vi "Documentation Application Tool.vi"() -> ()   [LabVIEW 2016]
uses:
  <vilib>/ni/Tree/Tree Manager/Tree.lvclass
  States.ctl
  <vilib>/ni/Tree/Data Types/String/String.lvclass/String.ctl
  <vilib>/ni/Tree/Data Types/String/To String Tree Data.vi
  <vilib>/ni/Tree/Data Types/String/From String Tree Data.vi
  <vilib>/ni/Tree/Data Types/String/String.lvclass
  C:/Program Files/National Instruments/LabVIEW 2016/vi.lib/ni/Tree/Tree Data/Tree Data.lvclass
  <vilib>/ni/Tree/Tree Manager/API/Set Meta Data.vi
  <vilib>/ni/Tree/Tree Manager/API/Set Attribute.vi
  <vilib>/ni/Tree/Tree Manager/API/Get Name.vi
  <vilib>/ni/Tree/Tree Manager/API/Set Name.vi
  <vilib>/ni/Tree/Tree Manager/API/Set Attribute Tree Data.vi
  <vilib>/xml/Load XML File.vi
  <vilib>/ni/Tree/Tree Manager/API/List Roots.vi
  <vilib>/ni/Tree/Tree Manager/API/Get Attribute Tree Data.vi
  <vilib>/ni/Tree/Tree Manager/API/Get Meta Data.vi
  <vilib>/ni/Tree/Tree Manager/API/Delete Attribute Tree Data.vi
  <vilib>/ni/Tree/Tree Manager/API/List Attribute Names.vi
  <vilib>/ni/Tree/Tree Manager/API/Get Attribute.vi
  <vilib>/xml/NI_XML.lvlib
panel:
  in  "Load XML File":bool
  in  "XML File Path":path=path "C:/Git/rfic-reference-design-libraries-csharp/CodeReport.xml"
  in  "Load Search Directory":bool
  in  "Search Directory":path=path "C:/Git/rf-adv-reference-design-libraries-labview/Source/SG"
  in  "Code Modules":string(tree)
  in  "XML File":string(tree)
  out "Selected Element":string
  in  "Element Description":string
  in  "Copy":bool
  out "Selected XML Data":string
  in  "Cancel":bool
  in  "Apply All Unsaved":bool
  in  "Cancel All":bool
  in  "Apply":bool
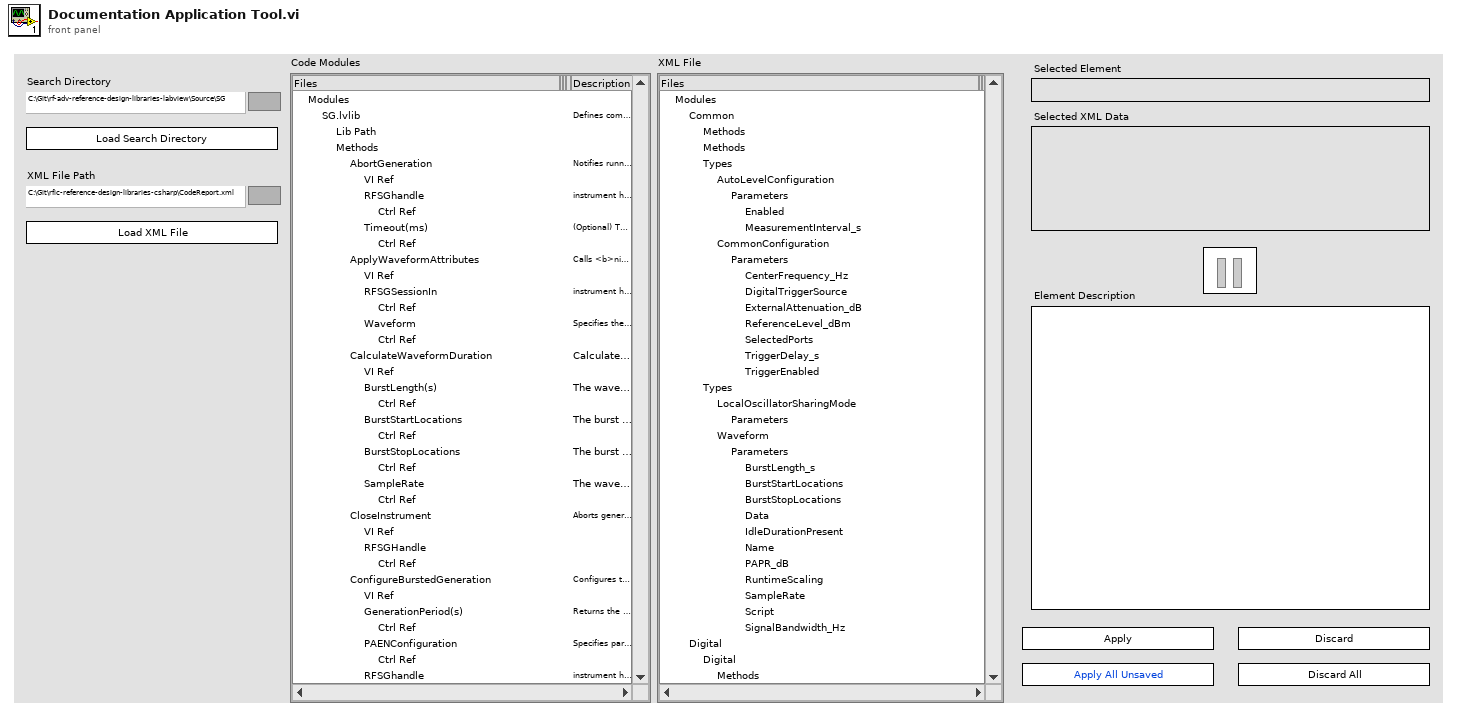
[diagram p1: front panel]
types:
  T1 = typedef "States.ctl" = enum16{"<Init>", "Wait for Event", "Update Code Modules Display", "Save Files", "<Shutdown>"}
  T2 = cluster{"LabVIEW Tree":refnum<data-value>, "XML Tree":refnum<data-value>, "References":refnum<vi>[], "Unsaved Items":variant, "Control Strings":string[], "Items to Save":string[]}
  T3 = enum32{"invalid VI type", "Standard VI", "Control VI", "Global VI", "Polymorphic VI", "Configuration VI", "SubSystem", "Facade VI", "Method VI", "Statechart Diagram VI"}
  T4 = enum16{"Left Button", "Center Button", "Right Button", "Window Close"}
  T5 = typedef "eventvkey.ctl" = enum16{"ASCII", "Enter", "Return", "Shift", "Ctrl", "Alt", "Cmd", "Opt", "Caps", "NumLock", "Clear", "Break", "Up", "Down", "Left", "Right", "Insert", "Delete", "Home", "End", "PageUp", "PageDown", "Escape", "Help", "Pause", "ScrollLock", "F1", "F2", "F3", "F4", "F5", "F6", "F7", "F8", "F9", "F10", "F11", "F12", "F13", "F14", "F15", "F16", "F17", "F18", "F19", "F20", "F21", "F22", "F23", "F24", "Play", "VolumeUp", "VolumeDown", "Mute", "Two Byte Char"}
  T6 = cluster{"Shift":bool, "Ctrl":bool, "Alt":bool, "Cmd":bool, "Opt":bool}
  T7 = cluster{"Left Cell String":string, "Child Text":string[], "Child Tag":string, "Item Indent":i32, "Child Only?":bool, "Glyph Index":i32}[]
  T8 = typedef "LVNodeAndColumnTypeDef.ctl" = cluster{"Node":string, "Column":i32}
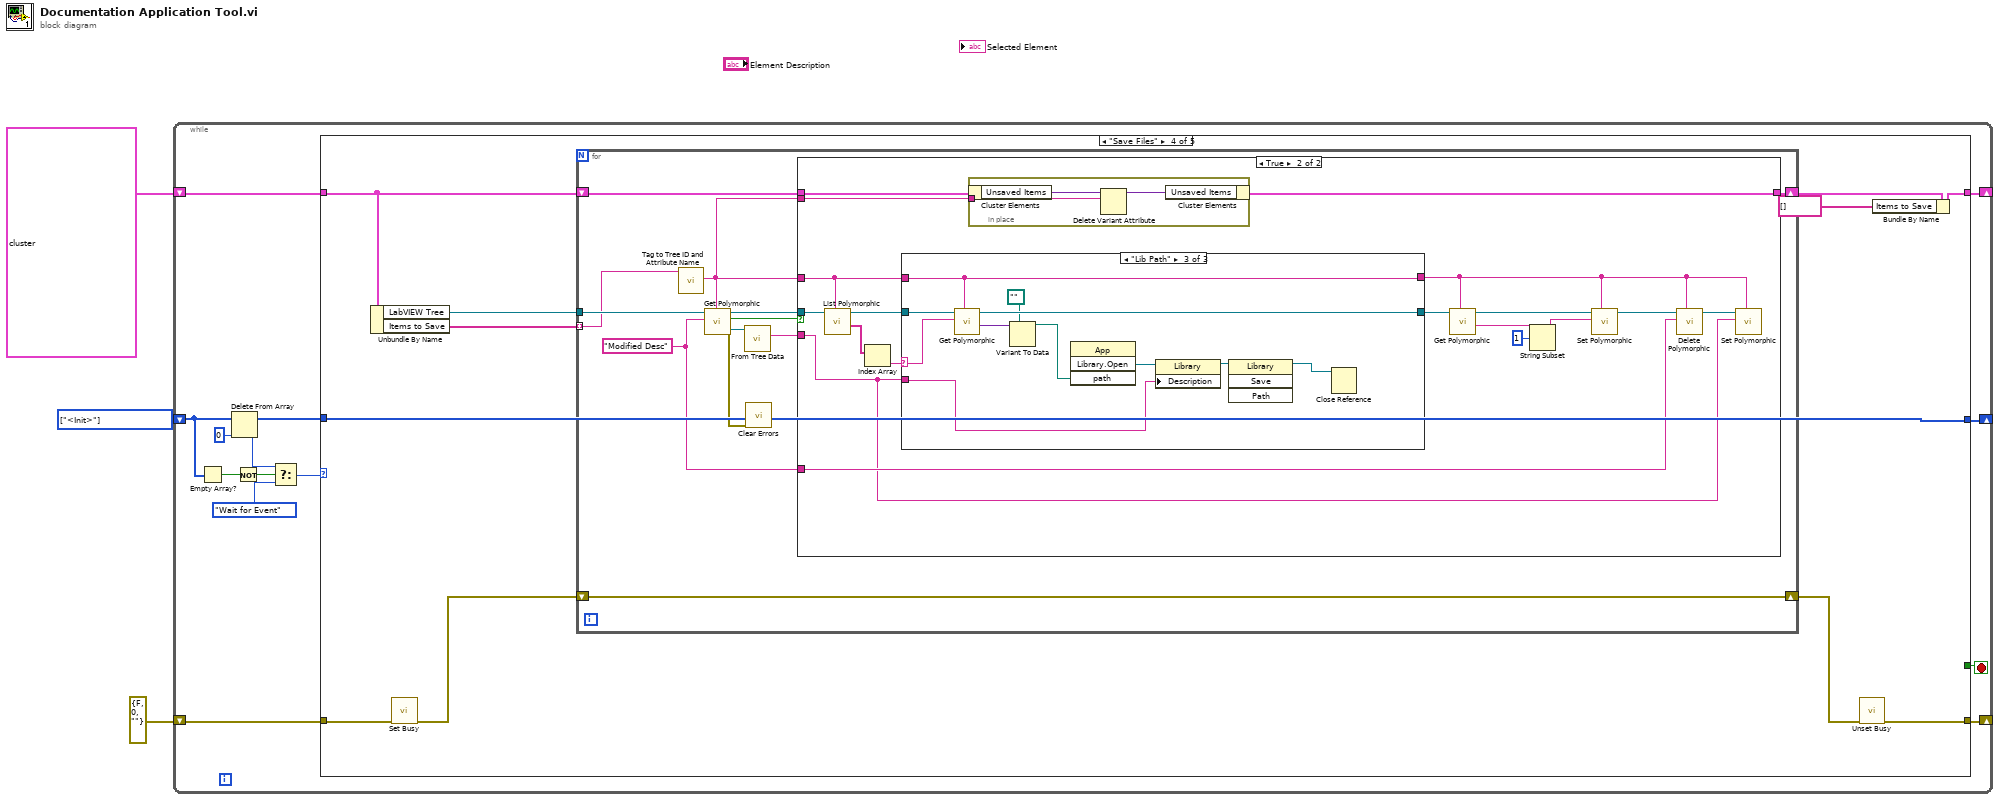
[diagram p0: block diagram]
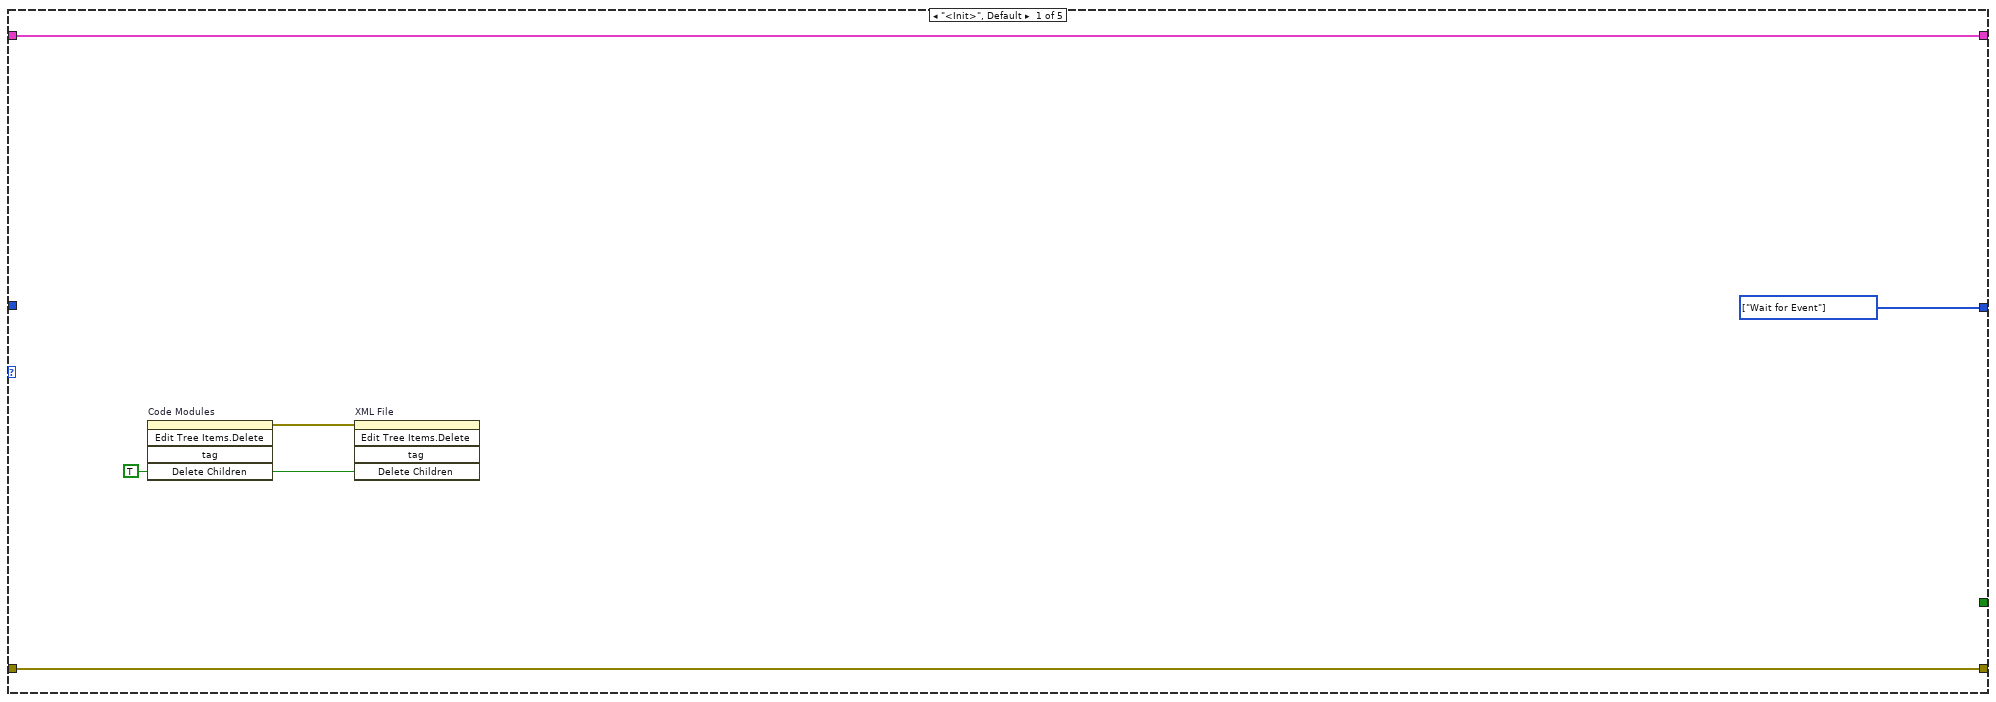
[diagram p2: hidden frame]
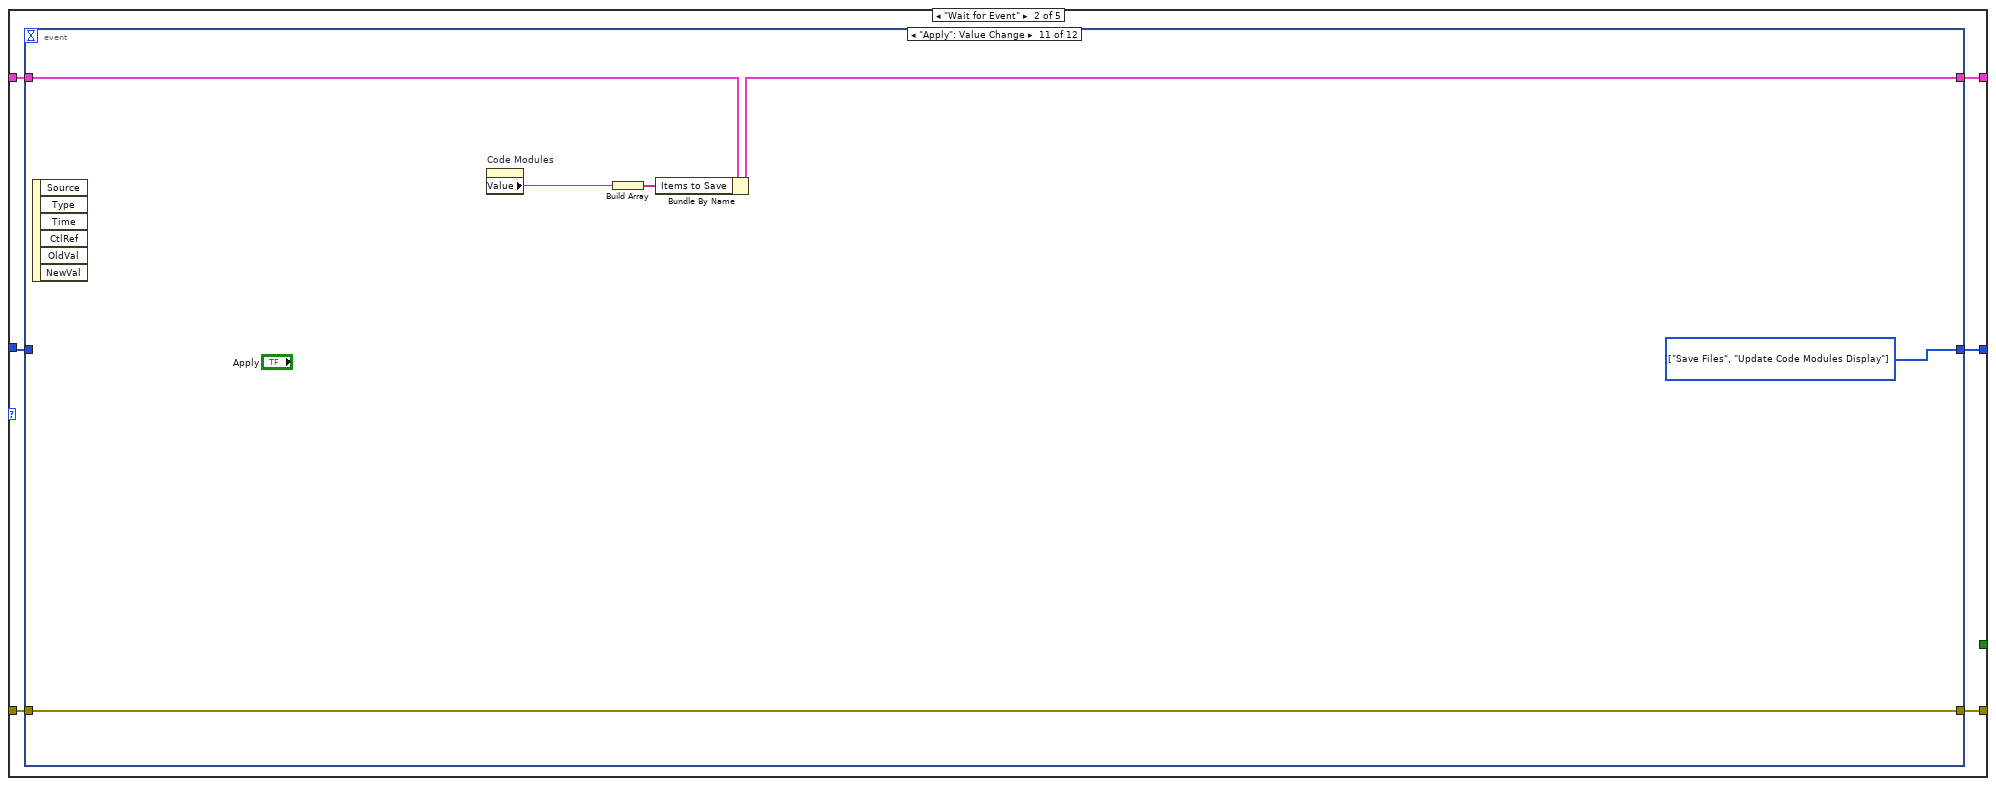
[diagram p3: hidden frame]
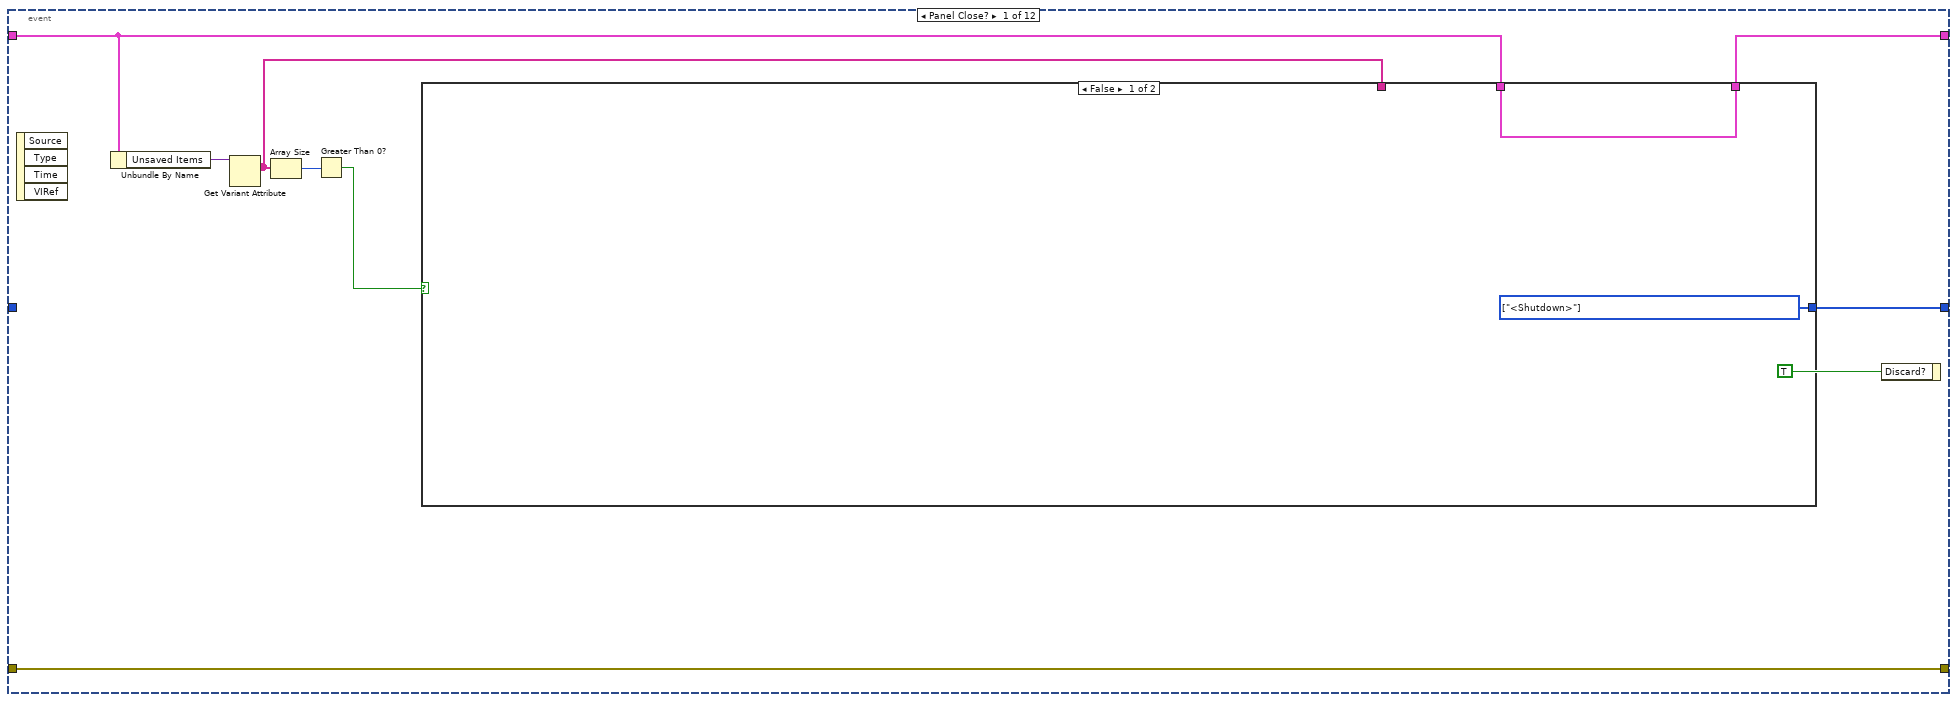
[diagram p4: hidden frame]
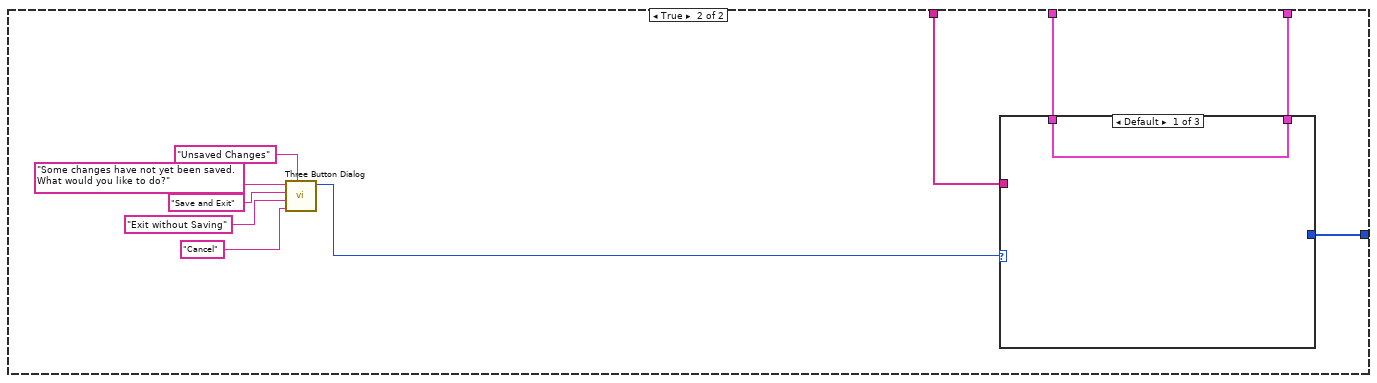
[diagram p5: hidden frame]
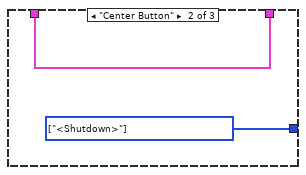
[diagram p6: hidden frame]
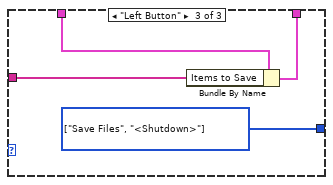
[diagram p7: hidden frame]
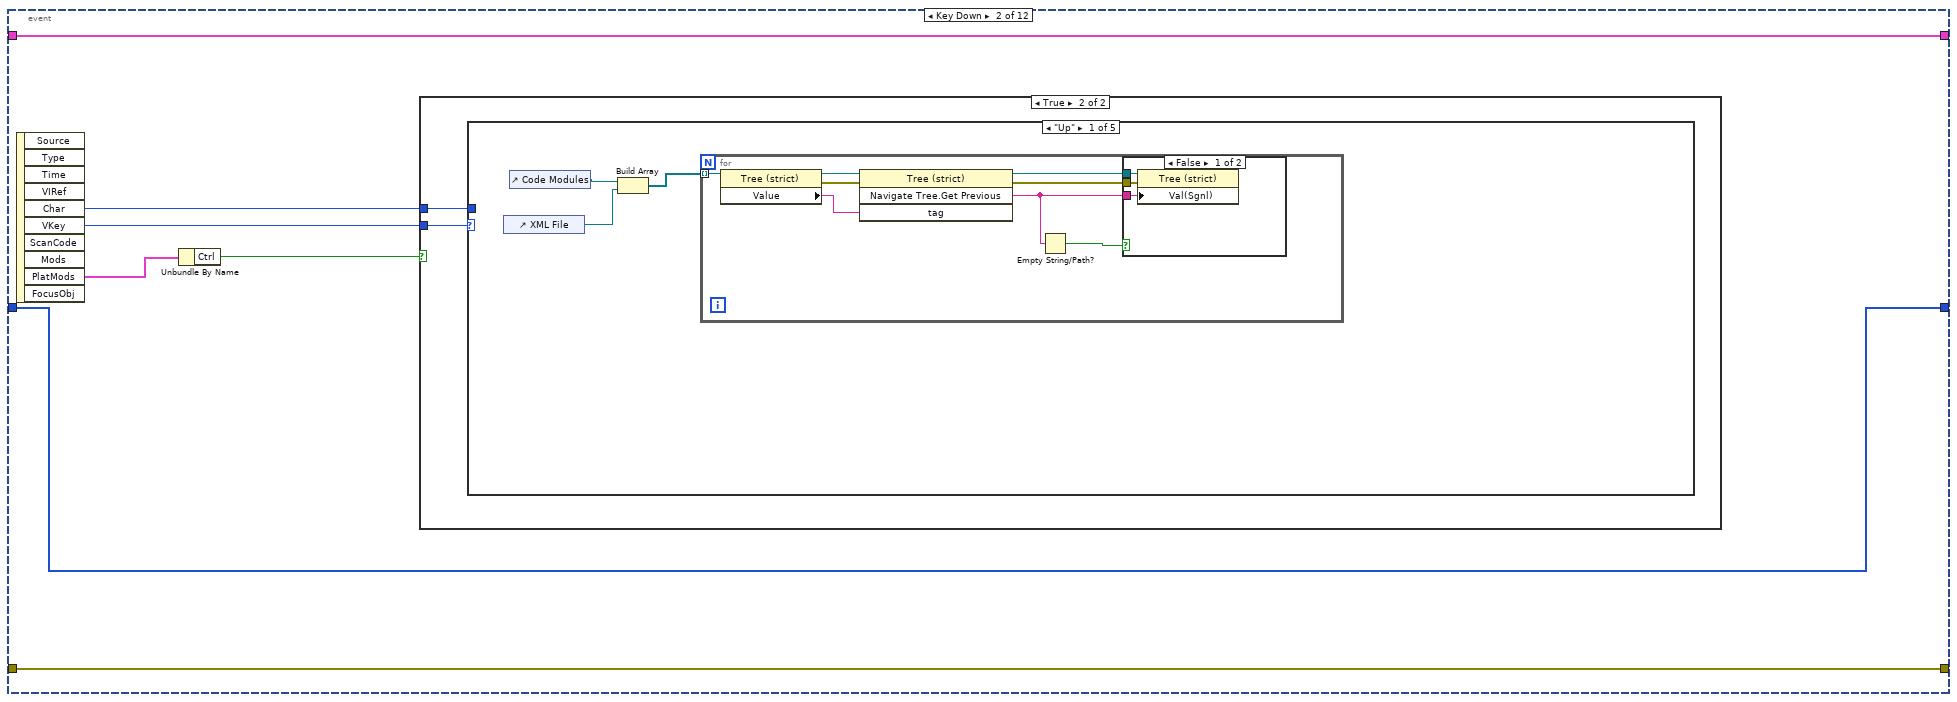
[diagram p8: hidden frame]
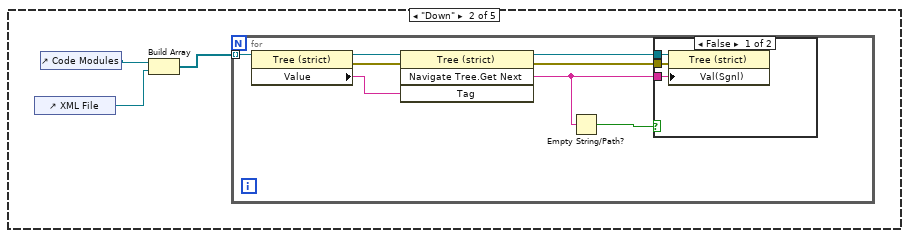
[diagram p11: hidden frame]
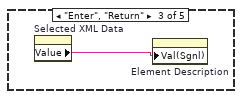
[diagram p13: hidden frame]
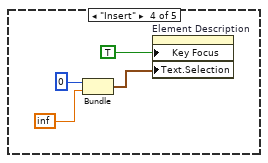
[diagram p14: hidden frame]
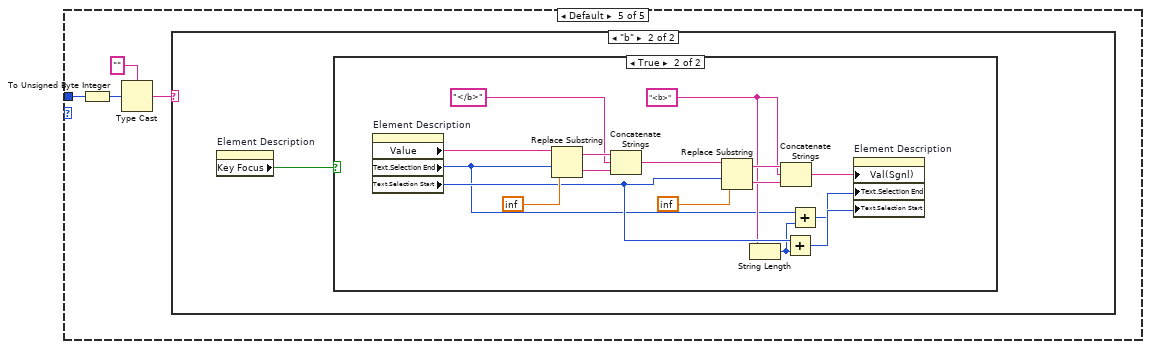
[diagram p15: hidden frame]
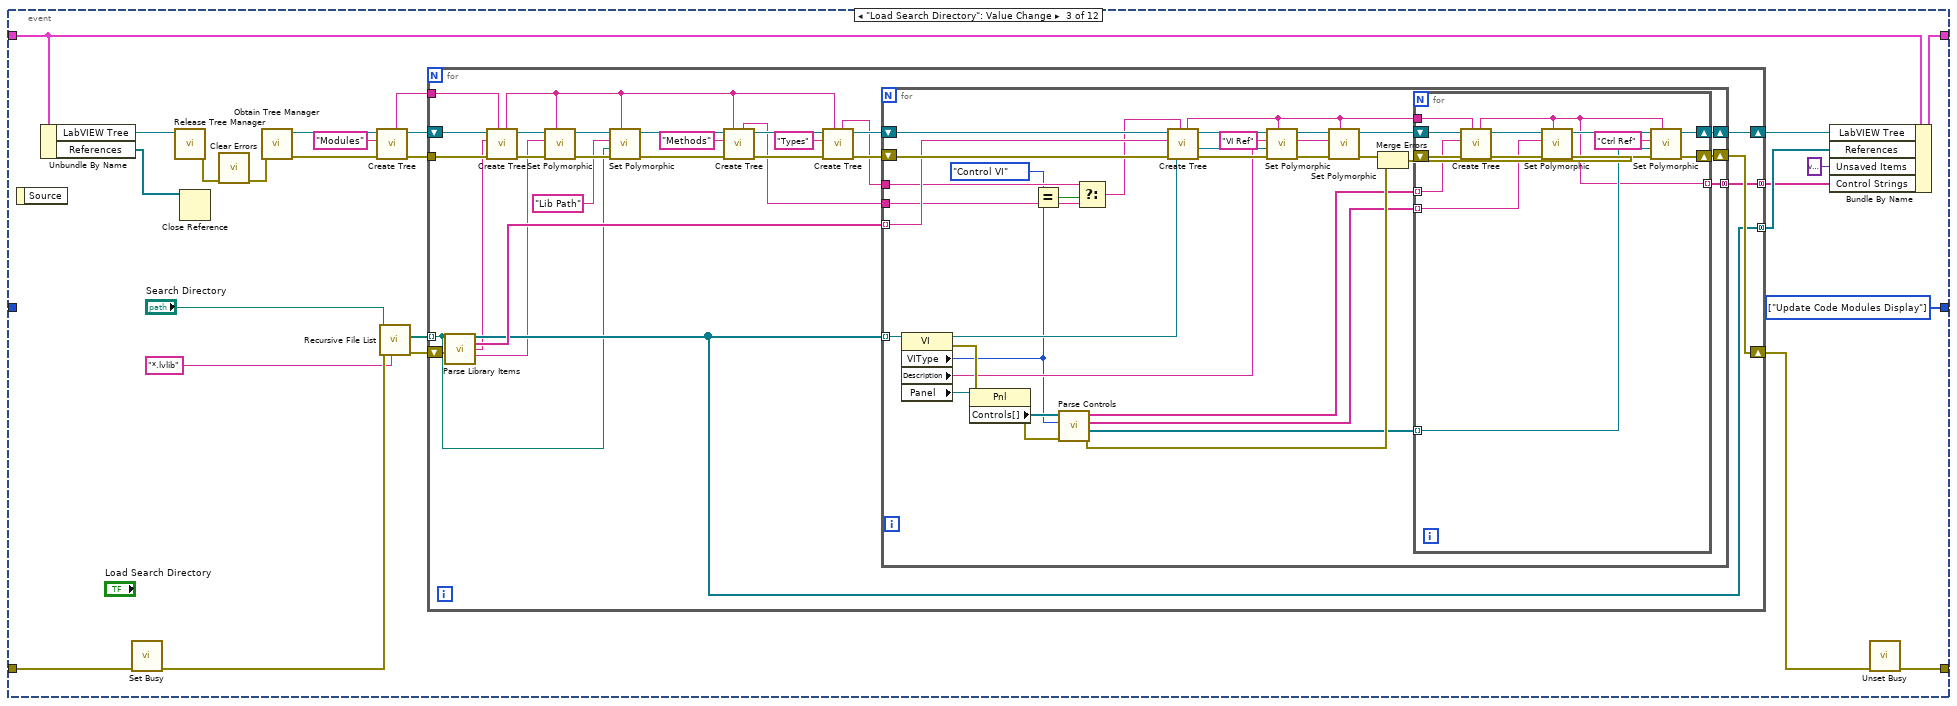
[diagram p18: hidden frame]
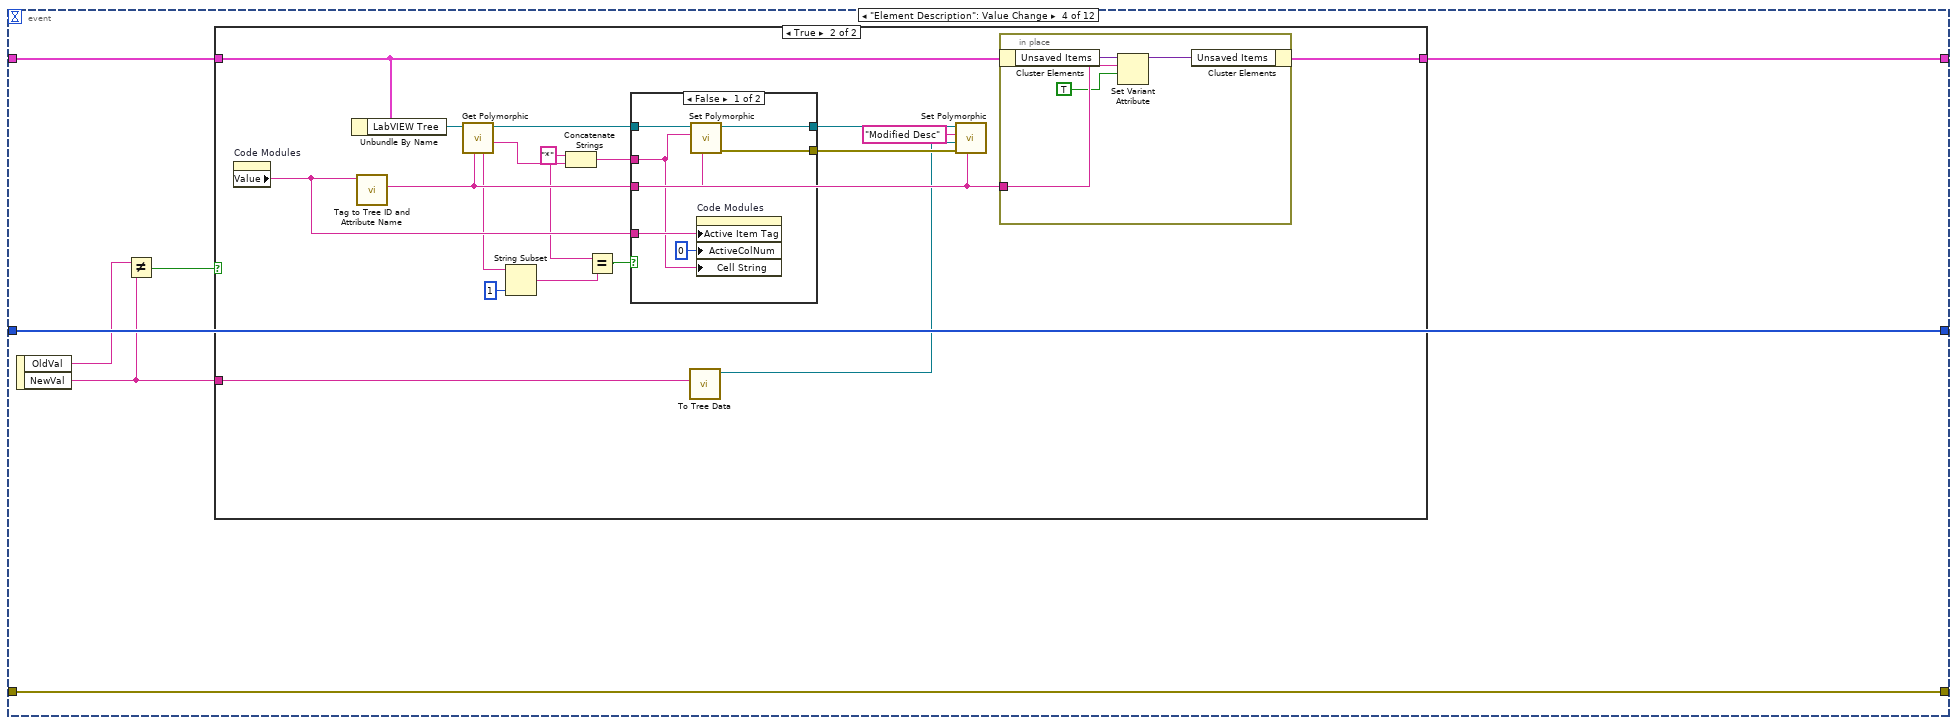
[diagram p19: hidden frame]
diagram:
  w1 = T1[] [enum."<Init>"] items=["<Init>", "Wait for Event", "Update Code Modules Display", "Save Files", "<Shutdown>"]
  n1 = while {
    shift-right: [w16] -> _
    shift-left: errorcluster {"status"=FALSE, "code"=0, "source"=""} ("error constant") -> [w17]
    shift-right: [w14] -> _
    shift-left: T2 {"LabVIEW Tree"=refnum, "XML Tree"=refnum, "References"=[], "Unsaved Items"=variant, "Control Strings"=[], "Items to Save"=[]} -> [w15]
    shift-right: [w5] -> _
    shift-left: w1 -> [w11]
    stop <- w4 stop-if-true
    n2 = Empty Array?(array=w11) -> (empty?=w10:bool)
    n3 = Delete From Array(array=w11, index=0) -> (deleted portion=w9:T1, array with subset deleted=w13:T1[])  [unwired: 1 in]
    n4 = Not(x=w10) -> (.not. x?=w8:bool)
    n5 = Select(t=w9, s=w8, f=States."Wait for Event") -> (s? t:f=w6:T1)
    n6 = case shown="\"Save Files\"" w6 {
      tunnel: w17 -> [w21 w28 w412 w439 w522]
      tunnel: [w21 w27 w412 w430 w522] -> w16
      tunnel: w15 -> [w18 w26 w405 w437 w519]
      tunnel: [w18 w25 w405 w434 w519] -> w14
      tunnel: w13 -> [_ w23 w388 w432 w520]
      tunnel: [w19 w24 w388 w432 w520] -> w5
      tunnel: [_ _ _ _ TRUE] -> w4
      frame "<Init>", Default {
        w19 = T1[] [enum."Wait for Event"] items=["<Init>", "Wait for Event", "Update Code Modules Display", "Save Files", "<Shutdown>"]
        w20 = TRUE ("Delete Children?")
        n7 = invoke on="Code Modules" class="Tree (strict)" method="Edit Tree Items.Delete"("Delete Children"=w20) -> (error out=w22:errorcluster)  [unwired: 4 in, 4 out]
        n8 = invoke on="XML File" class="Tree (strict)" method="Edit Tree Items.Delete"(error in=w22, "Delete Children"=w20) -> ()  [unwired: 3 in, 5 out]
      }
      frame "Wait for Event" {
        n9 = event shown="[10] \"Apply\": Value Change" {
          selector: _ -> [_ _ _ _ _ _ _ _ _ _ _ _]
          dyn-events: _ -> [_ _ _ _ _ _ _ _ _ _ _ _]
          timeout: _ -> [_ _ _ _ _ _ _ _ _ _ _ _]
          tunnel: w28 -> [w37 w63 w143 w225 w294 w298 w311 w318 w328 w355 w364 w370]
          tunnel: [w37 w63 w142 w225 w261 w298 w311 w318 w328 w355 w364 w370] -> w27
          tunnel: w26 -> [w32 w62 w126 w224 w280 w297 w310 w317 w327 w342 w362 w367]
          tunnel: [w31 w62 w127 w223 w281 w297 w310 w317 w320 w340 w361 w368] -> w25
          tunnel: [w35 w59 w123 w222 w263 w295 w299 w312 w325 w353 w363 w369] -> w24
          tunnel: w23 -> [_ w59 _ w222 w263 w295 w299 w312 _ _ _ _]
          event Panel Close? {
            n10 = event-data() -> ()  [unwired: 1 in, 4 out]
            n11 = Unbundle By Name(w32) -> ("Unsaved Items"=w34:variant)
            n12 = Get Variant Attribute(Variant=w34) -> (names=w30:string[])  [unwired: 3 in, 3 out]
            n13 = Array Size(array=w30) -> (size(s)=w33:i32)
            n14 = Greater Than 0?(x=w33) -> (x > 0?=w29:bool)
            n15 = case shown="False" w29 {
              tunnel: [w38 w49] -> w35
              tunnel: w32 -> [w39 w47]
              tunnel: [w39 w46] -> w31
              tunnel: w30 -> [_ w45]
              frame False {
                w38 = T1[] [enum."<Shutdown>"] items=["<Init>", "Wait for Event", "Update Code Modules Display", "Save Files", "<Shutdown>"]
              }
              frame True {
                n16 = call <vilib>:"Three Button Dialog.vi"("Window Title (\"\")"="Unsaved Changes" ("Window Title (\"\")"), "Right Button Text (\"Cancel\")"="Cancel" ("Right Button Text (\"Cancel\")"), "Center Button Text (\"No\")"="Exit without Saving" ("Center Button Text (\"No\")"), "Left Button Text (\"Yes\")"="Save and Exit" ("Left Button Text (\"Yes\")"), "message"="Some changes have not yet been saved. What would you like to do?") -> ("Which Button?"=w48:T4)  [unwired: 6 in]
                n17 = case shown="Default" w48 {
                  tunnel: [_ w52 w56] -> w49
                  tunnel: w47 -> [w50 w51 w55]
                  tunnel: [w50 w51 w54] -> w46
                  tunnel: w45 -> [_ _ w53]
                  frame Default {
                  }
                  frame "Center Button" {
                    w52 = T1[] [enum."<Shutdown>"] items=["<Init>", "Wait for Event", "Update Code Modules Display", "Save Files", "<Shutdown>"]
                  }
                  frame "Left Button" {
                    w56 = T1[] [enum."Save Files", enum."<Shutdown>"] items=["<Init>", "Wait for Event", "Update Code Modules Display", "Save Files", "<Shutdown>"]
                    n18 = Bundle By Name(cluster=w55, "Items to Save"=w53) -> (w54:T2)
                  }
                }
              }
            }
            n19 = event-data("Discard?"=TRUE) -> ()  [unwired: 1 in, 1 out]
          }
          event Key Down {
            n20 = event-data() -> ("Char"=w57:i16, "VKey"=w60:T5, "PlatMods"=w61:T6)  [unwired: 1 in, 7 out]
            n21 = Unbundle By Name(w61) -> ("Ctrl"=w58:bool)
            n22 = case shown="True" w58 {
              tunnel: w60 -> [_ w65]
              tunnel: w57 -> [_ w64]
              frame False {
              }
              frame True {
                n23 = case shown="\"Up\"" w65 {
                  tunnel: w64 -> [_ _ _ _ w102]
                  frame "Up" {
                    n24 = control-ref of="XML File"() -> (w67:refnum<vi>)
                    n25 = control-ref of="Code Modules"() -> (w68:refnum<vi>)
                    n26 = Build Array(w68, w67) -> (w66:refnum<vi>[])
                    n27 = for {
                      tunnel: w66 -> [w71] mode=indexing
                      n28 = property class="Tree (strict)"(reference=w71) -> (reference out=w74:refnum<vi>, error out=w73:errorcluster, "Value"=w76:string)  [unwired: 1 in]
                      n29 = invoke on="Invoke Node" class="Tree (strict)" method="Navigate Tree.Get Previous"(reference=w74, error in=w73, "tag"=w76) -> (reference out=w75:refnum<vi>, error out=w72:errorcluster, "Navigate Tree:Get Previous"=w70:string)  [unwired: 1 in, 1 out]
                      n30 = Empty String/Path?(string/path=w70) -> (empty?=w69:bool)
                      n31 = case shown="False" w69 {
                        tunnel: w75 -> [w79 _]
                        tunnel: w72 -> [w78 _]
                        tunnel: w70 -> [w77 _]
                        frame False {
                          n32 = property class="Tree (strict)"(reference=w79, error in=w78, "Val(Sgnl)"=w77) -> ()  [unwired: 2 out]
                        }
                        frame True {
                        }
                      }
                    }
                  }
                  frame "Down" {
                    n33 = control-ref of="XML File"() -> (w81:refnum<vi>)
                    n34 = control-ref of="Code Modules"() -> (w82:refnum<vi>)
                    n35 = Build Array(w82, w81) -> (w80:refnum<vi>[])
                    n36 = for {
                      tunnel: w80 -> [w85] mode=indexing
                      n37 = property class="Tree (strict)"(reference=w85) -> (reference out=w88:refnum<vi>, error out=w87:errorcluster, "Value"=w90:string)  [unwired: 1 in]
                      n38 = invoke on="Invoke Node" class="Tree (strict)" method="Navigate Tree.Get Next"(reference=w88, error in=w87, "Tag"=w90) -> (reference out=w89:refnum<vi>, error out=w86:errorcluster, "Navigate Tree:Get Next Item"=w84:string)  [unwired: 1 in, 1 out]
                      n39 = Empty String/Path?(string/path=w84) -> (empty?=w83:bool)
                      n40 = case shown="False" w83 {
                        tunnel: w89 -> [w93 _]
                        tunnel: w86 -> [w92 _]
                        tunnel: w84 -> [w91 _]
                        frame False {
                          n41 = property class="Tree (strict)"(reference=w93, error in=w92, "Val(Sgnl)"=w91) -> ()  [unwired: 2 out]
                        }
                        frame True {
                        }
                      }
                    }
                  }
                  frame "Enter", "Return" {
                    n42 = property on="Selected XML Data" class="Str"() -> ("Value"=w94:string)  [unwired: 2 in, 2 out]
                    n43 = property on="Element Description" class="Str"("Val(Sgnl)"=w94) -> ()  [unwired: 2 in, 2 out]
                  }
                  frame "Insert" {
                    n44 = Bundle(0, inf) -> (w95:cluster{i32, dbl})  [unwired: 1 in]
                    n45 = property on="Element Description" class="Str"("Key Focus"=TRUE, "Text.Selection"=w95) -> ()  [unwired: 2 in, 2 out]
                  }
                  frame Default {
                    n46 = To Unsigned Byte Integer(number=w102) -> (unsigned 8bit integer=w99:u8)
                    n47 = Type Cast(type="", x=w99) -> (*(type *) &x=w101:string)
                    n48 = case shown="\"b\"" w101 {
                      frame Default {
                      }
                      frame "b" {
                        n49 = property on="Element Description" class="Str"() -> ("Key Focus"=w103:bool)  [unwired: 2 in, 2 out]
                        n50 = case shown="True" w103 {
                          frame False {
                          }
                          frame True {
                            w108 = "<b>"
                            n51 = property on="Element Description" class="Str"() -> ("Value"=w119:string, "Text.Selection End"=w105:u32, "Text.Selection Start"=w109:u32)  [unwired: 2 in, 2 out]
                            n52 = Replace Substring(2:inf, 3:w105, 5:w119) -> (0:w117:string, 1:w118:string)  [unwired: 1 in]
                            n53 = Concatenate Strings(w118, "</b>", w117) -> (w113:string)
                            n54 = Replace Substring(2:inf, 3:w109, 5:w113) -> (0:w115:string, 1:w114:string)  [unwired: 1 in]
                            n55 = String Length(string=w108) -> (length=w106:i32)
                            n56 = Concatenate Strings(w114, w108, w115) -> (w112:string)
                            n57 = Add(x=w109, y=w106) -> (x+y=w107:u32)
                            n58 = Add(x=w105, y=w106) -> (x+y=w104:u32)
                            n59 = property on="Element Description" class="Str"("Val(Sgnl)"=w112, "Text.Selection End"=w104, "Text.Selection Start"=w107) -> ()  [unwired: 2 in, 2 out]
                          }
                        }
                      }
                    }
                  }
                }
              }
            }
          }
          event "Load Search Directory": Value Change {
            w123 = T1[] [enum."Update Code Modules Display"] items=["<Init>", "Wait for Event", "Update Code Modules Display", "Save Files", "<Shutdown>"]
            n60 = event-data() -> ()  [unwired: 1 in, 1 out]
            n61 = Unbundle By Name(w126) -> ("LabVIEW Tree"=w132:refnum<data-value>, "References"=w122:refnum<vi>[])
            n62 = call <vilib>:"Set Busy.vi"("error in (no error)"=w143) -> ("error out"=w137:errorcluster)  [unwired: 9 in, 1 out]
            n63 = call <vilib>:"Release Tree Manager.vi"("Tree"=w132) -> ("Error Out"=w141:errorcluster)  [unwired: 10 in]
            n64 = Close Reference(reference=w122) -> ()  [unwired: 1 in, 1 out]
            n65 = call <vilib>:"Clear Errors.vi"("error in (no error)"=w141) -> ("error out"=w140:errorcluster)  [unwired: 5 in, 1 out]
            n66 = call <vilib>:"Obtain Tree Manager.vi"("Error In"=w140) -> ("Error Out"=w139:errorcluster, "Tree"=w131:refnum<data-value>)  [unwired: 9 in]
            n67 = call <vilib>:"Create Tree.vi"("Error In"=w139, "Name"="Modules", "Tree Manager"=w131) -> ("Error Out"=w138:errorcluster, "Tree Manager"=w128:refnum<data-value>, "Unique ID"=w129:string)  [unwired: 6 in]
            n68 = call <vilib>:"Recursive File List.vi"("pattern"="*.lvlib", "error in (no error)"=w137, "Folder Path"="Search Directory") -> ("error out"=w144:errorcluster, "All Files in Dir"=w133:path[])  [unwired: 4 in, 3 out]
            n69 = for {
              tunnel: w133 -> [w147] mode=indexing
              shift-right: [w167] -> w136
              shift-left: w144 -> [w172]
              tunnel: w129 -> [w162]
              tunnel: w138 -> [w171]
              tunnel: [w165] -> w125 mode=concatenating
              shift-right: [w155] -> w124
              shift-left: w128 -> [w164]
              tunnel: [w154] -> w120 mode=concatenating
              n70 = call "Parse Library Items.vi"("Library Path"=w147, "error in (no error)"=w172) -> ("References"=w165:refnum<vi>[], "File Names"=w166:string[], "Display Name"=w163:string, "Description"=w151:string)  [unwired: 9 in, 1 out]
              n71 = call <vilib>:"Create Tree.vi"("Parent ID (empty)"=w162, "Error In"=w171, "Name"=w163, "Tree Manager"=w164) -> ("Error Out"=w170:errorcluster, "Tree Manager"=w152:refnum<data-value>, "Unique ID"=w145:string)  [unwired: 5 in]
              n72 = call-poly <vilib>:"Set Polymorphic.vi"("Tree ID"=w145, "Error In"=w170, "Meta Data"=w151, "Tree Manager"=w152) -> ("Error Out"=w153:errorcluster, "Tree Manager"=w149:refnum<data-value>)  [unwired: 6 in]
              n73 = call-poly <vilib>:"Set Polymorphic.vi"("Tree ID"=w145, "Error In"=w153, "Attribute Value"=w147, "Attribute Name"="Lib Path", "Tree Manager"=w149) -> ("Error Out"=w150:errorcluster, "Tree Manager"=w148:refnum<data-value>)  [unwired: 4 in, 1 out]
              n74 = call <vilib>:"Create Tree.vi"("Parent ID (empty)"=w145, "Error In"=w150, "Name"="Methods", "Tree Manager"=w148) -> ("Error Out"=w169:errorcluster, "Tree Manager"=w161:refnum<data-value>, "Unique ID"=w157:string)  [unwired: 5 in]
              n75 = call <vilib>:"Create Tree.vi"("Parent ID (empty)"=w145, "Error In"=w169, "Name"="Types", "Tree Manager"=w161) -> ("Error Out"=w168:errorcluster, "Tree Manager"=w158:refnum<data-value>, "Unique ID"=w156:string)  [unwired: 5 in]
              n76 = for {
                tunnel: w165 -> [w195] mode=indexing
                tunnel: w166 -> [w189] mode=indexing
                tunnel: w157 -> [w186]
                tunnel: w156 -> [w187]
                shift-right: [w176] -> w155
                shift-left: w158 -> [w190]
                shift-right: [w196] -> w167
                shift-left: w168 -> [w203]
                tunnel: [w173] -> w154 mode=concatenating
                n77 = property class="VI"(reference=w195) -> (reference out=w181:refnum<vi>, error out=w204:errorcluster, "VIType"=w174:T3, "Description"=w183:string, "Panel"=w175:refnum<vi>)  [unwired: 1 in]
                n78 = property class="Pnl"(reference=w175, error in=w204) -> (error out=w199:errorcluster, "Controls[]"=w194:refnum<vi>[])  [unwired: 1 out]
                n79 = Equal?(x=T3."Control VI" ("y"), y=w174) -> (x = y?=w188:bool)
                n80 = call "Parse Controls.vi"("error in (no error)"=w199, "VI Type"=w174, "Controls[]"=w194) -> ("error out"=w197:errorcluster, "References"=w191:refnum<vi>[], "Control Descriptions"=w192:string[], "Control Names"=w193:string[])  [unwired: 5 in]
                n81 = Select(t=w187, s=w188, f=w186) -> (s? t:f=w184:string)
                n82 = call <vilib>:"Create Tree.vi"("Parent ID (empty)"=w184, "Error In"=w203, "Name"=w189, "Tree Manager"=w190) -> ("Error Out"=w202:errorcluster, "Tree Manager"=w180:refnum<data-value>, "Unique ID"=w177:string)  [unwired: 5 in]
                n83 = call-poly <vilib>:"Set Polymorphic.vi"("Tree ID"=w177, "Error In"=w202, "Attribute Value"=w181, "Attribute Name"="VI Ref", "Tree Manager"=w180) -> ("Error Out"=w201:errorcluster, "Tree Manager"=w179:refnum<data-value>)  [unwired: 4 in, 1 out]
                n84 = call-poly <vilib>:"Set Polymorphic.vi"("Tree ID"=w177, "Error In"=w201, "Meta Data"=w183, "Tree Manager"=w179) -> ("Error Out"=w200:errorcluster, "Tree Manager"=w178:refnum<data-value>)  [unwired: 6 in]
                n85 = Merge Errors(w200, w197) -> (w198:errorcluster)
                n86 = for {
                  tunnel: w193 -> [w212] mode=indexing
                  tunnel: w192 -> [w211] mode=indexing
                  tunnel: w191 -> [w206] mode=indexing
                  shift-right: [w215] -> w196
                  shift-left: w198 -> [w218]
                  tunnel: w177 -> [w213]
                  shift-right: [w208] -> w176
                  shift-left: w178 -> [w214]
                  tunnel: [w205] -> w173 mode=indexing
                  n87 = call <vilib>:"Create Tree.vi"("Parent ID (empty)"=w213, "Error In"=w218, "Name"=w212, "Tree Manager"=w214) -> ("Error Out"=w217:errorcluster, "Tree Manager"=w210:refnum<data-value>, "Unique ID"=w205:string)  [unwired: 5 in]
                  n88 = call-poly <vilib>:"Set Polymorphic.vi"("Tree ID"=w205, "Error In"=w217, "Meta Data"=w211, "Tree Manager"=w210) -> ("Error Out"=w216:errorcluster, "Tree Manager"=w209:refnum<data-value>)  [unwired: 6 in]
                  n89 = call-poly <vilib>:"Set Polymorphic.vi"("Tree ID"=w205, "Error In"=w216, "Attribute Value"=w206, "Attribute Name"="Ctrl Ref", "Tree Manager"=w209) -> ("Error Out"=w215:errorcluster, "Tree Manager"=w208:refnum<data-value>)  [unwired: 4 in, 1 out]
                }
              }
            }
            n90 = Bundle By Name(cluster=w126, "LabVIEW Tree"=w124, "References"=w125, "Unsaved Items"=variant, "Control Strings"=w120) -> (w127:T2)
            n91 = call <vilib>:"Unset Busy.vi"("error in (no error)"=w136) -> ("error out"=w142:errorcluster)  [unwired: 10 in]
          }
          event "Element Description": Value Change {
            n92 = event-data() -> ("OldVal"=w219:string, "NewVal"=w220:string)  [unwired: 1 in]
            n93 = Not Equal?(x=w219, y=w220) -> (x != y?=w221:bool)
            n94 = case shown="True" w221 {
              tunnel: w224 -> [w226 w239]
              tunnel: [w226 w238] -> w223
              tunnel: w220 -> [_ w234]
              frame False {
              }
              frame True {
                w228 = "*" ("string")
                n95 = property on="Code Modules" class="Tree (strict)"() -> ("Value"=w240:string)  [unwired: 2 in, 2 out]
                n96 = Unbundle By Name(w239) -> ("LabVIEW Tree"=w242:refnum<data-value>)
                n97 = call <vilib>:"Tag to Tree ID and Attribute Name.vi"("Tag"=w240) -> ("Tree ID"=w236:string)  [unwired: 8 in, 2 out]
                n98 = call-poly <vilib>:"Get Polymorphic.vi"("Tree ID"=w236, "Tree Manager"=w242) -> ("Name"=w232:string, "Tree Manager"=w241:refnum<data-value>)  [unwired: 7 in, 1 out]
                n99 = String Subset(string=w232, length (rest)=1 ("length (rest)")) -> (substring=w229:string)  [unwired: 1 in]
                n100 = Concatenate Strings(w228, w232) -> (w230:string)
                n101 = Equal?(x=w228, y=w229) -> (x = y?=w227:bool)
                n102 = case shown="False" w227 {
                  tunnel: [w250 _] -> w243
                  tunnel: w241 -> [w249 w251]
                  tunnel: w240 -> [w248 _]
                  tunnel: [w246 w251] -> w237
                  tunnel: w236 -> [w245 _]
                  tunnel: w230 -> [w244 _]
                  frame False {
                    n103 = call-poly <vilib>:"Set Polymorphic.vi"("Tree ID"=w245, "Name"=w244, "Tree Manager"=w249) -> ("Error Out"=w250:errorcluster, "Tree Manager"=w246:refnum<data-value>)  [unwired: 7 in]
                    n104 = property on="Code Modules" class="Tree (strict)"("Active Item Tag"=w248, "ActiveColNum"=0 ("Active Cell:Active Column Number"), "Cell String"=w244) -> ()  [unwired: 2 in, 2 out]
                  }
                  frame True {
                  }
                }
                n105 = call-poly <vilib>:"To Tree Data.vi"("String"=w234) -> ("String Tree Data"=w233:refnum<class "String.lvclass">)  [unwired: 10 in]
                n106 = call-poly <vilib>:"Set Polymorphic.vi"("Tree ID"=w236, "Error In"=w243, "Attribute Value"=w233, "Attribute Name"="Modified Desc", "Tree Manager"=w237) -> ()  [unwired: 4 in, 3 out]
                n107 = in-place {
                  in-place-border: w236 -> [w254]
                  n108 = in-place-cluster #1(w239) -> ("Unsaved Items"=w255:variant)
                  n109 = Set Variant Attribute(Variant=w255, name=w254, value=TRUE) -> (Variant out=w253:variant)  [unwired: 1 in, 2 out]
                  n110 = in-place-cluster #1("Unsaved Items"=w253) -> (w238:T2)
                }
              }
            }
          }
          event "Load XML File": Value Change {
            n111 = event-data() -> ()  [unwired: 1 in, 1 out]
            n112 = call <vilib>:"Set Busy.vi"("error in (no error)"=w294) -> ("error out"=w262:errorcluster)  [unwired: 9 in, 1 out]
            n113 = Unbundle By Name(w280) -> ("XML Tree"=w283:refnum<data-value>)
            n114 = call <vilib>:"Release Tree Manager.vi"("Error In"=w262, "Tree"=w283) -> ("Error Out"=w293:errorcluster)  [unwired: 9 in]
            n115 = control-ref of="XML File"() -> (w264:refnum<vi>)
            n116 = call <vilib>:"Clear Errors.vi"("error in (no error)"=w293) -> ("error out"=w292:errorcluster)  [unwired: 5 in, 1 out]
            n117 = call <vilib>:"Obtain Tree Manager.vi"("Error In"=w292) -> ("Error Out"=w290:errorcluster, "Tree"=w282:refnum<data-value>)  [unwired: 9 in]
            n118 = property class="Tree (strict)"(reference=w264) -> (reference out=w272:refnum<vi>, error out=w286:errorcluster, "OwningVI"=w270:refnum<vi>)  [unwired: 1 in]
            n119 = call-poly <vilib>:"Load.vi"("path to XML document"="XML File Path", "error in (no error)"=w290) -> ("DOM document out"=w278:refnum<k20>, "error out"=w291:errorcluster)  [unwired: 11 in, 1 out]
            n120 = call "Recursive XML Parse - Specific.vi"("error in (no error)"=w291, "DOM document in"=w278, "Tree"=w282) -> ("Tree Manager"=w268:refnum<data-value>)  [unwired: 7 in, 1 out]
            n121 = property class="VI"(reference=w270, error in=w286) -> (error out=w287:errorcluster, "Panel"=w271:refnum<vi>)  [unwired: 1 out]
            n122 = property class="Pnl"(reference=w271, error in=w287, "DeferPanUpdts"=TRUE ("Defer Panel Updates")) -> (reference out=w276:refnum<vi>, error out=w288:errorcluster)
            n123 = invoke class="Tree (strict)" method="Edit Tree Items.Delete"(reference=w272, error in=w288) -> (reference out=w275:refnum<vi>, error out=w284:errorcluster)  [unwired: 3 in, 3 out]
            n124 = call-poly <vilib>:"List Polymorphic.vi"("Error In"=w284, "Tree"=w268) -> ("Error Out"=w285:errorcluster, "Tree"=w267:refnum<data-value>, "Roots IDs"=w266:string[])  [unwired: 6 in, 1 out]
            n125 = Index Array(array=w266) -> (element=w265:string)  [unwired: 1 in]
            n126 = call <vilib>:"Show Tree.vi"("Root ID"=w265, "Error In"=w285, "Tree"=w267) -> ("Error Out"=w289:errorcluster, "Items Out"=w277:T7, "Tree"=w269:refnum<data-value>)  [unwired: 6 in]
            n127 = invoke class="Tree (strict)" method="Edit Tree Items.Add Multiple Items to End"(reference=w275, error in=w289, "Items"=w277) -> (reference out=w257:refnum<vi>, error out=w259:errorcluster)  [unwired: 1 in, 2 out]
            n128 = Bundle By Name(cluster=w280, "XML Tree"=w269) -> (w281:T2)
            n129 = invoke class="Tree (strict)" method="Edit Tree Items.Sort Children"(reference=w257, error in=w259, "Sort Recursively"=TRUE ("Sort Recursively?")) -> (error out=w258:errorcluster)  [unwired: 5 in, 7 out]
            n130 = property class="Pnl"(reference=w276, error in=w258, "DeferPanUpdts"=FALSE ("Defer Panel Updates")) -> (error out=w260:errorcluster)  [unwired: 1 out]
            n131 = call <vilib>:"Unset Busy.vi"("error in (no error)"=w260) -> ("error out"=w261:errorcluster)  [unwired: 10 in]
          }
          event "Copy": Value Change {
            n132 = event-data() -> ()  [unwired: 1 in, 6 out]
            n133 = property on="Selected XML Data" class="Str"() -> ("Value"=w296:string)  [unwired: 2 in, 2 out]
            n134 = property on="Element Description" class="Str"("Val(Sgnl)"=w296) -> ()  [unwired: 2 in, 2 out]
          }
          event "Code Modules": Value Change {
            # "Get modified description if existing"
            n135 = event-data() -> ("NewVal"=w309:string)  [unwired: 1 in, 4 out]
            n136 = Unbundle By Name(w310) -> ("LabVIEW Tree"=w302:refnum<data-value>)
            n137 = call <vilib>:"Tag to Tree ID and Attribute Name.vi"("Tag"=w309) -> ("Tree ID"=w306:string)  [unwired: 8 in, 2 out]
            n138 = call-poly <vilib>:"Get Polymorphic.vi"("Tree ID"=w306, "Attribute Name"="Modified Desc", "Tree Manager"=w302) -> ("Error Out"=w300:errorcluster, "Attribute Value"=w308:refnum<class "Tree Data.lvclass">, "Found?"=w305:bool)  [unwired: 5 in, 1 out]
            n139 = call-poly <vilib>:"Get Polymorphic.vi"("Tree ID"=w306, "Tree Manager"=w302) -> ("Meta Data"=w303:string)  [unwired: 7 in, 2 out]
            n140 = call <vilib>:"Clear Errors.vi"("error in (no error)"=w300) -> ()  [unwired: 5 in, 2 out]
            n141 = call-poly <vilib>:"From Tree Data.vi"("Tree Data"=w308) -> ("String"=w304:string)  [unwired: 10 in]
            n142 = Select(t=w304, s=w305, f=w303) -> (s? t:f=w301:string)
            n143 = property on="Element Description" class="Str"("Value"=w301) -> ()  [unwired: 2 in, 2 out]
          }
          event "XML File": Value Change {
            n144 = event-data() -> ("NewVal"=w313:string)  [unwired: 1 in, 4 out]
            n145 = Unbundle By Name(w317) -> ("XML Tree"=w316:refnum<data-value>)
            n146 = call <vilib>:"Tag to Tree ID and Attribute Name.vi"("Tag"=w313) -> ("Tree ID"=w315:string)  [unwired: 8 in, 2 out]
            n147 = call-poly <vilib>:"Get Polymorphic.vi"("Tree ID"=w315, "Tree Manager"=w316) -> ("Meta Data"=→"Selected XML Data":string)  [unwired: 7 in, 2 out]
          }
          event "Cancel All": Value Change {
            w325 = T1[] [enum."Update Code Modules Display"] items=["<Init>", "Wait for Event", "Update Code Modules Display", "Save Files", "<Shutdown>"]
            n148 = event-data() -> ()  [unwired: 1 in, 6 out]
            n149 = Unbundle By Name(w327) -> ("Unsaved Items"=w322:variant, "LabVIEW Tree"=w326:refnum<data-value>)
            n150 = Get Variant Attribute(Variant=w322) -> (names=w321:string[])  [unwired: 3 in, 3 out]
            n151 = for {
              tunnel: w321 -> [w332] mode=indexing
              tunnel: w326 -> [w337]
              tunnel: [w329] -> w323
              n152 = call-poly <vilib>:"Get Polymorphic.vi"("Tree ID"=w332, "Tree Manager"=w337) -> ("Error Out"=w338:errorcluster, "Name"=w335:string, "Tree Manager"=w336:refnum<data-value>)  [unwired: 7 in]
              n153 = String Subset(string=w335, offset (0)=1) -> (substring=w334:string)  [unwired: 1 in]
              n154 = call-poly <vilib>:"Set Polymorphic.vi"("Tree ID"=w332, "Error In"=w338, "Name"=w334, "Tree Manager"=w336) -> ("Error Out"=w339:errorcluster, "Tree Manager"=w331:refnum<data-value>)  [unwired: 6 in]
              n155 = call-poly <vilib>:"Delete Polymorphic.vi"("Tree ID"=w332, "Error In"=w339, "Attribute Name"="Modified Desc", "Tree Manager"=w331) -> ("Error Out"=w329:errorcluster)  [unwired: 4 in, 3 out]
            }
            n156 = property on="Code Modules" class="Tree (strict)"(error in=w323) -> ("Value"=w324:string)  [unwired: 1 in, 2 out]
            n157 = property on="Code Modules" class="Tree (strict)"("Val(Sgnl)"=w324) -> ()  [unwired: 2 in, 2 out]
            n158 = Bundle By Name(cluster=w327, "Unsaved Items"=variant) -> (w320:T2)
          }
          event "Cancel": Value Change {
            w353 = T1[] [enum."Update Code Modules Display"] items=["<Init>", "Wait for Event", "Update Code Modules Display", "Save Files", "<Shutdown>"]
            n159 = event-data() -> ()  [unwired: 1 in, 6 out]
            n160 = property on="Code Modules" class="Tree (strict)"() -> ("Value"=w341:string)  [unwired: 2 in, 2 out]
            n161 = Unbundle By Name(w342) -> ("LabVIEW Tree"=w354:refnum<data-value>)
            n162 = in-place {
              in-place-border: w341 -> [w356]
              n163 = in-place-cluster #2(w342) -> ("Unsaved Items"=w358:variant)
              n164 = Delete Variant Attribute(6:w356, 7:w358) -> (3:w357:variant)  [unwired: 1 in, 2 out]
              n165 = in-place-cluster #2("Unsaved Items"=w357) -> (w340:T2)
            }
            n166 = call-poly <vilib>:"Get Polymorphic.vi"("Tree ID"=w341, "Tree Manager"=w354) -> ("Error Out"=w349:errorcluster, "Name"=w347:string, "Tree Manager"=w348:refnum<data-value>)  [unwired: 7 in]
            n167 = String Subset(string=w347, offset (0)=1) -> (substring=w346:string)  [unwired: 1 in]
            n168 = call-poly <vilib>:"Set Polymorphic.vi"("Tree ID"=w341, "Error In"=w349, "Name"=w346, "Tree Manager"=w348) -> ("Error Out"=w350:errorcluster, "Tree Manager"=w344:refnum<data-value>)  [unwired: 6 in]
            n169 = call-poly <vilib>:"Delete Polymorphic.vi"("Tree ID"=w341, "Error In"=w350, "Attribute Name"="Modified Desc", "Tree Manager"=w344) -> ("Error Out"=w351:errorcluster)  [unwired: 4 in, 3 out]
            n170 = property on="Code Modules" class="Tree (strict)"(error in=w351) -> ("Value"=w352:string)  [unwired: 1 in, 2 out]
            n171 = property on="Code Modules" class="Tree (strict)"("Val(Sgnl)"=w352) -> ()  [unwired: 2 in, 2 out]
          }
          event "Apply": Value Change {
            w363 = T1[] [enum."Save Files", enum."Update Code Modules Display"] items=["<Init>", "Wait for Event", "Update Code Modules Display", "Save Files", "<Shutdown>"]
            n172 = event-data() -> ()  [unwired: 1 in, 6 out]
            n173 = property on="Code Modules" class="Tree (strict)"() -> ("Value"=w360:string)  [unwired: 2 in, 2 out]
            n174 = Build Array(w360) -> (w359:string[])
            n175 = Bundle By Name(cluster=w362, "Items to Save"=w359) -> (w361:T2)
          }
          event "Apply All Unsaved": Value Change {
            w369 = T1[] [enum."Save Files", enum."Update Code Modules Display"] items=["<Init>", "Wait for Event", "Update Code Modules Display", "Save Files", "<Shutdown>"]
            n176 = event-data() -> ()  [unwired: 1 in, 6 out]
            n177 = Unbundle By Name(w367) -> ("Unsaved Items"=w366:variant)
            n178 = Get Variant Attribute(Variant=w366) -> (names=w365:string[])  [unwired: 3 in, 3 out]
            n179 = Bundle By Name(cluster=w367, "Items to Save"=w365) -> (w368:T2)
          }
        }
      }
      frame "Update Code Modules Display" {
        n180 = control-ref of="Code Modules"() -> (w392:refnum<vi>)
        n181 = call <vilib>:"Set Busy.vi"() -> ("error out"=w379:errorcluster)  [unwired: 10 in, 1 out]
        n182 = property class="Tree (strict)"(reference=w392, error in=w379) -> (reference out=w387:refnum<vi>, error out=w408:errorcluster, "OwningVI"=w398:refnum<vi>)
        n183 = Unbundle By Name(w405) -> ("Control Strings"=w389:string[], "LabVIEW Tree"=w395:refnum<data-value>)
        n184 = property class="Tree (strict)"(reference=w387) -> (reference out=w385:refnum<vi>, error out=w371:errorcluster, "All Tags"=w386:string[], "TopLeft"=w373:T8)  [unwired: 1 in]
        n185 = property class="VI"(reference=w398, error in=w408) -> (error out=w409:errorcluster, "Panel"=w399:refnum<vi>)  [unwired: 1 out]
        n186 = call <vilib>:"Clear Errors.vi"("error in (no error)"=w371) -> ()  [unwired: 5 in, 2 out]
        n187 = for {
          tunnel: w386 -> [w422] mode=indexing
          tunnel: [w421] -> w380 mode=indexing
          shift-right: [w419] -> w384
          shift-left: w385 -> [w419]
          n188 = property class="Tree (strict)"(reference=w419, "Active Item Tag"=w422) -> ("Open?"=w420:bool)  [unwired: 1 in, 2 out]
          n189 = Bundle(w422, "Open?"=w420) -> (w421:cluster{string, "Open?":bool})  [unwired: 1 in]
        }
        n190 = property class="Pnl"(reference=w399, error in=w409, "DeferPanUpdts"=TRUE ("Defer Panel Updates")) -> (reference out=w403:refnum<vi>, error out=w410:errorcluster)
        n191 = invoke class="Tree (strict)" method="Edit Tree Items.Delete"(reference=w384, error in=w410, "Delete Children"=TRUE ("Delete Children?")) -> (reference out=w402:refnum<vi>, error out=w376:errorcluster)  [unwired: 2 in, 3 out]
        n192 = call-poly <vilib>:"List Polymorphic.vi"("Error In"=w376, "Tree"=w395) -> ("Error Out"=w407:errorcluster, "Tree"=w396:refnum<data-value>, "Roots IDs"=w397:string[])  [unwired: 6 in, 1 out]
        n193 = Index Array(array=w397) -> (element=w394:string)  [unwired: 1 in]
        n194 = call <vilib>:"Show Tree.vi"("Root ID"=w394, "Error In"=w407, "Tree"=w396) -> ("Error Out"=w411:errorcluster, "Items Out"=w404:T7)  [unwired: 6 in, 1 out]
        n195 = invoke class="Tree (strict)" method="Edit Tree Items.Add Multiple Items to End"(reference=w402, error in=w411, "Items"=w404) -> (reference out=w393:refnum<vi>, error out=w406:errorcluster)  [unwired: 1 in, 2 out]
        n196 = invoke on="Invoke Node" class="Tree (strict)" method="Edit Tree Items.Sort Children"(reference=w393, error in=w406) -> (reference out=w391:refnum<vi>, error out=w390:errorcluster)  [unwired: 6 in, 6 out]
        n197 = for {
          tunnel: w390 -> [w427]
          tunnel: w389 -> [w426] mode=indexing
          tunnel: [w424] -> w382
          shift-right: [w423] -> w383
          shift-left: w391 -> [w428]
          n198 = invoke on="Invoke Node" class="Tree (strict)" method="Open/Close.Item"(reference=w428, error in=w427, "tag"=w426, "Open"=FALSE ("Open?")) -> (reference out=w423:refnum<vi>, error out=w424:errorcluster)  [unwired: 1 in, 3 out]
        }
        n199 = for {
          tunnel: [w417] -> w381
          tunnel: w382 -> [w417]
          tunnel: w380 -> [w416] mode=indexing
          shift-right: [w418] -> w374
          shift-left: w383 -> [w418]
          n200 = Unbundle(w416) -> (w415:string, "Open?"=w414:bool)
          n201 = property class="Tree (strict)"(reference=w418, "Active Item Tag"=w415, "Open?"=w414) -> (error out=w413:errorcluster)  [unwired: 1 in, 1 out]
          n202 = call <vilib>:"Clear Errors.vi"("error in (no error)"=w413) -> ()  [unwired: 5 in, 2 out]
        }
        n203 = property class="Tree (strict)"(reference=w374, error in=w381, "TopLeft"=w373) -> (error out=w375:errorcluster)  [unwired: 1 out]
        n204 = call <vilib>:"Clear Errors.vi"("error in (no error)"=w375) -> ("error out"=w372:errorcluster)  [unwired: 5 in, 1 out]
        n205 = property class="Pnl"(reference=w403, error in=w372, "DeferPanUpdts"=FALSE ("Defer Panel Updates")) -> (error out=w378:errorcluster)  [unwired: 1 out]
        n206 = call <vilib>:"Unset Busy.vi"("error in (no error)"=w378) -> ()  [unwired: 10 in, 1 out]
      }
      frame "Save Files" {
        n207 = Unbundle By Name(w437) -> ("LabVIEW Tree"=w438:refnum<data-value>, "Items to Save"=w435:string[])
        n208 = call <vilib>:"Set Busy.vi"("error in (no error)"=w439) -> ("error out"=w431:errorcluster)  [unwired: 9 in, 1 out]
        n209 = for {
          tunnel: w438 -> [w451]
          shift-right: [w442] -> w436
          shift-left: w437 -> [w443]
          tunnel: w435 -> [w441] mode=indexing
          shift-right: [w440] -> w429
          shift-left: w431 -> [w440]
          w444 = "Modified Desc" ("Attribute Name")
          n210 = call <vilib>:"Tag to Tree ID and Attribute Name.vi"("Tag"=w441) -> ("Tree ID"=w445:string)  [unwired: 8 in, 2 out]
          n211 = call-poly <vilib>:"Get Polymorphic.vi"("Tree ID"=w445, "Attribute Name"=w444, "Tree Manager"=w451) -> ("Error Out"=w450:errorcluster, "Attribute Value"=w447:refnum<class "Tree Data.lvclass">, "Found?"=w449:bool, "Tree Manager"=w448:refnum<data-value>)  [unwired: 5 in]
          n212 = call-poly <vilib>:"From Tree Data.vi"("Tree Data"=w447) -> ("String"=w446:string)  [unwired: 10 in]
          n213 = call <vilib>:"Clear Errors.vi"("error in (no error)"=w450) -> ()  [unwired: 5 in, 2 out]
          n214 = case shown="True" w449 {
            tunnel: w448 -> [_ w457]
            tunnel: w446 -> [_ w460]
            tunnel: w443 -> [w452 w470]
            tunnel: [w452 w469] -> w442
            tunnel: w445 -> [_ w468]
            tunnel: w445 -> [_ w456]
            tunnel: w444 -> [_ w462]
            frame False {
            }
            frame True {
              n215 = call-poly <vilib>:"List Polymorphic.vi"("Tree ID"=w456, "Tree Manager"=w457) -> ("Attribute Names"=w454:string[], "Tree Manager"=w455:refnum<data-value>)  [unwired: 7 in, 1 out]
              n216 = Index Array(array=w454) -> (element=w453:string)  [unwired: 1 in]
              n217 = case shown="\"Lib Path\"" w453 {
                selector: w453 -> [_ w475 w505]
                tunnel: w460 -> [_ w480 w500]
                tunnel: w456 -> [w472 w474 w507]
                tunnel: [w472 w479 w507] -> w459
                tunnel: w455 -> [w471 w478 w508]
                tunnel: [w471 w477 w506] -> w458
                frame Default {
                }
                frame "Ctrl Ref", "VI Ref" {
                  n218 = call-poly <vilib>:"Get Polymorphic.vi"("Tree ID"=w474, "Attribute Name"=w475, "Tree Manager"=w478) -> ("Attribute Value"=w473:variant, "Tree Manager"=w476:refnum<data-value>)  [unwired: 5 in, 2 out]
                  n219 = case shown="\"Ctrl Ref\"" w475 {
                    tunnel: [w484 w496] -> w482
                    tunnel: w480 -> [w485 w495]
                    tunnel: [w489 w492] -> w479
                    tunnel: w474 -> [w489 w492]
                    tunnel: w476 -> [w483 w491]
                    tunnel: [w483 w491] -> w477
                    tunnel: w473 -> [w488 w490]
                    frame "Ctrl Ref" {
                      n220 = Variant To Data(type=refnum<vi> refnum ("References"), Variant=w488) -> (data=w486:refnum<vi>)  [unwired: 1 in, 1 out]
                      n221 = property class="Ctl"(reference=w486, "Desc"=w485) -> ("OwningVI"=w484:refnum<vi>)  [unwired: 1 in, 2 out]
                    }
                    frame "VI Ref", Default {
                      n222 = Variant To Data(type=refnum<vi> refnum ("reference out"), Variant=w490) -> (data=w493:refnum<vi>)  [unwired: 1 in, 1 out]
                      n223 = property class="VI"(reference=w493, "Description"=w495) -> (reference out=w496:refnum<vi>)  [unwired: 1 in, 1 out]
                    }
                  }
                  n224 = Not A Number/Path/Refnum?(number/path/refnum=w482) -> (NaN/Path/Refnum?=w481:bool)
                  n225 = case shown="False" w481 {
                    tunnel: w482 -> [w497 _]
                    frame False {
                      n226 = invoke class="VI" method="Save.Instrument"(reference=w497) -> ()  [unwired: 5 in, 6 out]
                    }
                    frame True {
                    }
                  }
                }
                frame "Lib Path" {
                  n227 = call-poly <vilib>:"Get Polymorphic.vi"("Tree ID"=w507, "Attribute Name"=w505, "Tree Manager"=w508) -> ("Attribute Value"=w504:variant, "Tree Manager"=w506:refnum<data-value>)  [unwired: 5 in, 2 out]
                  n228 = Variant To Data(type=path "", Variant=w504) -> (data=w502:path)  [unwired: 1 in, 1 out]
                  n229 = invoke class="App" method="Library.Open"("path"=w502) -> ("Open Library"=w501:refnum<vi>)  [unwired: 3 in, 3 out]
                  n230 = property class="Library"(reference=w501, "Description"=w500) -> (reference out=w499:refnum<vi>)  [unwired: 1 in, 1 out]
                  n231 = invoke class="Library" method="Save"(reference=w499) -> (reference out=w498:refnum<vi>)  [unwired: 3 in, 3 out]
                  n232 = Close Reference(reference=w498) -> ()  [unwired: 1 in, 1 out]
                }
              }
              n233 = in-place {
                in-place-border: w468 -> [w509]
                n234 = in-place-cluster #3(w470) -> ("Unsaved Items"=w511:variant)
                n235 = Delete Variant Attribute(6:w509, 7:w511) -> (3:w510:variant)  [unwired: 1 in, 2 out]
                n236 = in-place-cluster #3("Unsaved Items"=w510) -> (w469:T2)
              }
              n237 = call-poly <vilib>:"Get Polymorphic.vi"("Tree ID"=w459, "Tree Manager"=w458) -> ("Name"=w465:string, "Tree Manager"=w467:refnum<data-value>)  [unwired: 7 in, 1 out]
              n238 = String Subset(string=w465, offset (0)=1) -> (substring=w464:string)  [unwired: 1 in]
              n239 = call-poly <vilib>:"Set Polymorphic.vi"("Tree ID"=w459, "Name"=w464, "Tree Manager"=w467) -> ("Tree Manager"=w463:refnum<data-value>)  [unwired: 7 in, 1 out]
              n240 = call-poly <vilib>:"Delete Polymorphic.vi"("Tree ID"=w459, "Attribute Name"=w462, "Tree Manager"=w463) -> ("Tree Manager"=w461:refnum<data-value>)  [unwired: 5 in, 3 out]
              n241 = call-poly <vilib>:"Set Polymorphic.vi"("Tree ID"=w459, "Meta Data"=w460, "Tree Manager"=w461) -> ()  [unwired: 7 in, 2 out]
            }
          }
        }
        n242 = call <vilib>:"Unset Busy.vi"("error in (no error)"=w429) -> ("error out"=w430:errorcluster)  [unwired: 10 in]
        n243 = Bundle By Name(cluster=w436, "Items to Save"=string[] []) -> (w434:T2)
      }
      frame "<Shutdown>" {
        n244 = Unbundle By Name(w519) -> ("LabVIEW Tree"=w513:refnum<data-value>, "XML Tree"=w512:refnum<data-value>, "References"=w514:refnum<vi>[])
        n245 = call <vilib>:"Release Tree Manager.vi"("Tree"=w513) -> ("Error Out"=w518:errorcluster)  [unwired: 10 in]
        n246 = call <vilib>:"Release Tree Manager.vi"("Tree"=w512) -> ("Error Out"=w517:errorcluster)  [unwired: 10 in]
        n247 = Close Reference(reference=w514) -> (error out=w516:errorcluster)  [unwired: 1 in]
        n248 = Merge Errors(w518, w517, w516) -> (w515:errorcluster)
        n249 = call <vilib>:"Clear Errors.vi"("error in (no error)"=w515) -> ()  [unwired: 5 in, 2 out]
      }
    }
  }
